vi "Begin.vi"(8 "error in":errorcluster) -> (0 "error out":errorcluster)   [LabVIEW 2018]
doc: "Called before other user functions, this VI is expected to open initial I/O refnums, load in file data, and do all program initialization. Notice that the <B>error out</B> terminal is simply used for data flow. Wiring it to other structures or subVIs ensures that this VI runs first."
uses:
  <vilib>/Rock Robotics/SystemInterfaces/DIO/FPGA_DIOPWMChannel.ctl
  <vilib>/Rock Robotics/WPI/DriverStation/WPI_DriverStationRobotMode2.ctl
  <vilib>/Rock Robotics/WPI/Joystick/WPI_JoystickDeviceEnum.ctl
  <vilib>/Rock Robotics/WPI/Solenoid/WPI_SolenoidChannel.ctl
  <vilib>/Rock Robotics/SystemInterfaces/DIO/FPGA_DIOChannel.ctl
  <vilib>/Rock Robotics/WPI/SafetyOutput/WPI_SafetyOutputConfigMenu.ctl
  Robot Global Data.vi
  <vilib>/Rock Robotics/Network Tables/NT Write String Array.vi
  <vilib>/Rock Robotics/WPI/RobotDrive/WPI_RobotDriveOpen4MotorWithTalonSRX.vi
  <vilib>/Rock Robotics/WPI/Solenoid/WPI_SolenoidOpenSingle.vi
  <vilib>/Rock Robotics/WPI/Switch/WPI_SwitchOpenLimit.vi
  <vilib>/Rock Robotics/WPI/MotorControl/WPI_MotorControlOpen TalonSRX.vi
  Global 1.vi
  <vilib>/Rock Robotics/WPI/Counter/WPI_CounterDigitalInputToDigitalSource.vi
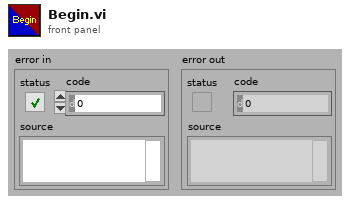
[diagram p1: front panel]
types:
  T1 = typedef "FPGA_DIOChannel.ctl" = enum8{"DIO 0", "DIO 1", "DIO 2", "DIO 3", "DIO 4", "DIO 5", "DIO 6", "DIO 7", "DIO 8", "DIO 9", "DIO MXP 0", "DIO MXP 1", "DIO MXP 2", "DIO MXP 3", "DIO MXP 4", "DIO MXP 5", "DIO MXP 6", "DIO MXP 7", "DIO MXP 8", "DIO MXP 9", "DIO MXP 10", "DIO MXP 11", "DIO MXP 12", "DIO MXP 13", "DIO MXP 14", "DIO MXP 15", "SPI Port CS1", "SPI Port CS2", "SPI Port CS3", "SPI Port MISO", "SPI Port MOSI", "Invalid"}
  T2 = typedef "WPI_SafetyOutputConfigMenu.ctl" = enum16{"Enable", "Disable"}
  T3 = typedef "FPGA_DIOPWMChannel.ctl" = enum8{"PWM 0", "PWM 1", "PWM 2", "PWM 3", "PWM 4", "PWM 5", "PWM 6", "PWM 7", "PWM 8", "PWM 9", "PWM MXP 0", "PWM MXP 1", "PWM MXP 2", "PWM MXP 3", "PWM MXP 4", "PWM MXP 5", "PWM MXP 6", "PWM MXP 7", "PWM MXP 8", "PWM MXP 9", "Invalid"}
  T4 = typedef "WPI_JoystickDeviceEnum.ctl" = enum16{"USB 0", "USB 1", "USB 2", "USB 3", "USB 4", "USB 5"}
  T5 = typedef "WPI_SolenoidChannel.ctl" = enum8{"Solenoid 0", "Solenoid 1", "Solenoid 2", "Solenoid 3", "Solenoid 4", "Solenoid 5", "Solenoid 6", "Solenoid 7", "Invalid"}
  T6 = typedef "WPI_DriverStationRobotMode2.ctl" = enum16{"Autonomous Disabled", "Autonomous Enabled", "Teleop Disabled", "Teleop Enabled", "Disconnected", "Finish", "Test Disabled", "Test Enabled", "Emergency Stopped"}
  T7 = typedef "WPI_MotorControlDeviceRef.ctl" = cluster{"DeviceStatus":errorcluster, "Type":T8, "PWM":cluster{"PWM Channel":T3, "DeadBand":T9}, "CAN":cluster{"Device Number":u8, "SetOutput VI Ref":variant, "GetOutput VI Ref":variant, "Enable VI Ref":variant, "Disable VI Ref":variant, "Data":variant}, "Invert":bool, "DIO PWM":cluster{"PWM \"Enable\" Channel":T3, "DIOChannel":T1, "PWM Rate":dbl}}
  T8 = typedef "WPI_MotorControlType.ctl" = enum16{"PWM", "CAN", "DIO PWM"}
  T9 = typedef "WPI_PWMDeadband.ctl" = cluster{"Name":string, "maxPositivePwm":i32, "minPositivePwm":i32, "centerPwm":i32, "maxNegativePwm":i32, "minNegativePwm":i32, "angularRange":u16}
  T10 = typedef "WPI_RobotDriveDevRef.ctl" = cluster{"DevStatus":errorcluster, "Motors[]":T7[], "Square Inputs":bool, "Max Output":dbl}
  T11 = typedef "WPI_JoystickDevRef.ctl" = cluster{"Device":T4}
  T12 = typedef "WPI_DigitalInputDevRef.ctl" = cluster{"DevStatus":errorcluster, "DIO Channel":T1}
  T13 = typedef "FPGA_CounterEncoderSourceConvertionLVSourceType.ctl" = cluster{"DevStatus":errorcluster, "AnalogTriggerMode?":bool, "DigitalMode":cluster{"DIO Channel":T14}, "AnalogTriggerMode":cluster{"AnalogTriggerIndex":T15, "OutputType":T16}}
  T14 = typedef "FPGA_DIODigitalSourceChannel.ctl" = enum8{"DIO 0", "DIO 1", "DIO 2", "DIO 3", "DIO 4", "DIO 5", "DIO 6", "DIO 7", "DIO 8", "DIO 9", "DIO MXP 0", "DIO MXP 1", "DIO MXP 2", "DIO MXP 3", "DIO MXP 4", "DIO MXP 5", "DIO MXP 6", "DIO MXP 7", "DIO MXP 8", "DIO MXP 9", "DIO MXP 10", "DIO MXP 11", "DIO MXP 12", "DIO MXP 13", "DIO MXP 14", "DIO MXP 15", "SPI Port CS1", "SPI Port CS2", "SPI Port CS3", "SPI Port MISO", "SPI Port MOSI", "Disabled"}
  T15 = typedef "FPGA_AnalogTriggerIndex.ctl" = enum8{"Trig 0", "Trig 1", "Trig 2", "Trig 3", "Trig 4", "Trig 5", "Trig 6", "Trig 7", "Invalid"}
  T16 = typedef "FPGA_AnalogTriggerOutType.ctl" = enum16{"InWindow", "TriggerState", "Rising", "Falling"}
  T17 = typedef "WPI_SolenoidDevRef.ctl" = cluster{"DevStatus":errorcluster, "Pneumatics Control Module":u8, "Forward Solenoid Channel":T5, "Reverse Solenoid Channel":T5}
  T18 = typedef "WPI_EncoderDevRef.ctl" = cluster{"DevStatus":errorcluster, "EncoderIndex":T19, "CounterIndex":T20, "DistancePerCount":dbl, "Decoding Type":T21}
  T19 = typedef "FPGA_EncoderIdx.ctl" = enum8{"Enc 0", "Enc 1", "Enc 2", "Enc 3", "Enc 4", "Enc 5", "Enc 6", "Enc 7", "Invalid"}
  T20 = typedef "FPGA_CounterCtrSystemIndex.ctl" = enum8{"Ctr 0", "Ctr 1", "Ctr 2", "Ctr 3", "Ctr 4", "Ctr 5", "Ctr 6", "Ctr 7", "Invalid"}
  T21 = typedef "WPI_EncoderType.ctl" = enum16{"1x", "2x", "4x"}
  T22 = typedef "WPI_SwitchDevRef.ctl" = cluster{"DevStatus":errorcluster, "DIO Channel":T1, "CntIndex":T20, "Normally Closed":bool}
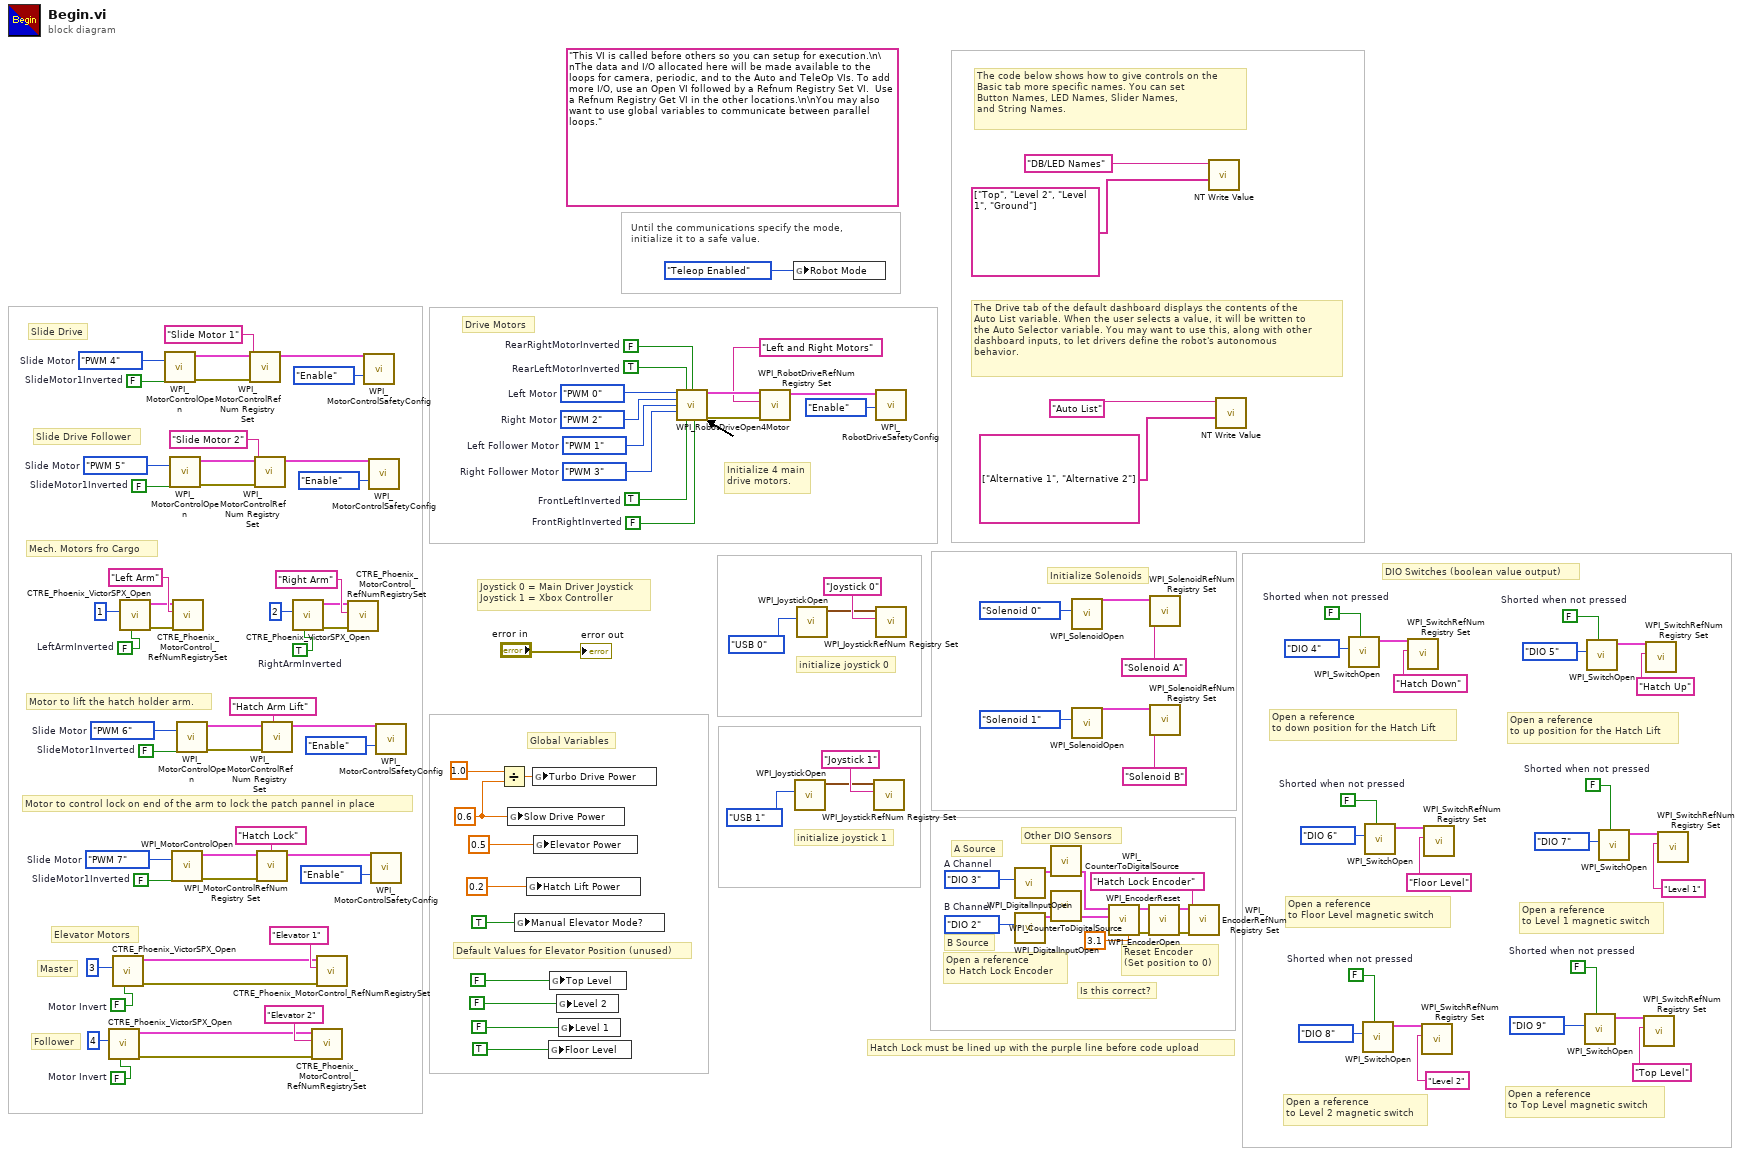
[diagram p0: block diagram]
diagram:
  w19 = FPGA_DIOChannel."DIO 2"  # B Channel
  w18 = FPGA_DIOChannel."DIO 3"  # A Channel
  w21 = FALSE  # Shorted when not pressed
  w25 = FALSE  # Shorted when not pressed
  w31 = FALSE  # SlideMotor1Inverted
  w36 = FPGA_DIOPWMChannel."PWM 7"  # Slide Motor
  w38 = FALSE  # SlideMotor1Inverted
  w43 = FPGA_DIOPWMChannel."PWM 6"  # Slide Motor
  w1 = FALSE  # Motor Invert
  w54 = FALSE  # SlideMotor1Inverted
  w60 = FPGA_DIOPWMChannel."PWM 5"  # Slide Motor
  w53 = TRUE  # RightArmInverted
  w49 = FALSE  # LeftArmInverted
  w63 = 0.6
  w44 = FALSE  # Motor Invert
  w73 = FALSE  # Shorted when not pressed
  w76 = FALSE  # SlideMotor1Inverted
  w82 = FPGA_DIOPWMChannel."PWM 4"  # Slide Motor
  w85 = FALSE  # Shorted when not pressed
  w86 = FALSE  # Shorted when not pressed
  w87 = FALSE  # Shorted when not pressed
  w104 = TRUE  # FrontLeftInverted
  w105 = FALSE  # FrontRightInverted
  w106 = FPGA_DIOPWMChannel."PWM 3"  # Right Follower Motor
  w107 = FPGA_DIOPWMChannel."PWM 1"  # Left Follower Motor
  (unwired) "This VI is called before others so you can setup for execution.\n\nThe data and I/O allocated here will be made available to the loops for camera, periodic, and to the Auto and TeleOp VIs. To add more I/O, use an Open VI followed by a Refnum Registry Set VI.  Use a Refnum Registry Get VI in the other locations.\n\nYou may also want to use global variables to communicate between parallel loops."
  w119 = FPGA_DIOPWMChannel."PWM 2"  # Right Motor
  w120 = FPGA_DIOPWMChannel."PWM 0"  # Left Motor
  w124 = TRUE  # RearLeftMotorInverted
  w125 = FALSE  # RearRightMotorInverted
  # "B Source"
  # "A Source"
  # "Hatch Lock must be lined up with the purple line before code upload"
  # "Is this correct?"
  # "Reset Encoder\n(Set position to 0)"
  # "Open a reference\nto Hatch Lock Encoder"
  # "Other DIO Sensors"
  # "DIO Switches (boolean value output)"
  # "Open a reference\nto up position for the Hatch Lift"
  # "Open a reference\nto down position for the Hatch Lift"
  # "Default Values for Elevator Position (unused)"
  # "Elevator Motors"
  # "Motor to control lock on end of the arm to lock the patch pannel in place"
  # "Motor to lift the hatch holder arm."
  # "Global Variables"
  # "Follower"
  # "Master"
  # "Slide Drive Follower"
  # "Slide Drive"
  # "Open a reference\nto Top Level magnetic switch"
  # "Drive Motors"
  # "Mech. Motors fro Cargo"
  # "Open a reference\nto Level 2 magnetic switch"
  # "Open a reference\nto Level 1 magnetic switch"
  # "Open a reference\nto Floor Level magnetic switch"
  # "Initialize Solenoids"
  # "Initialize 4 main\ndrive motors."
  # "Joystick 0 = Main Driver Joystick\nJoystick 1 = Xbox Controller"
  # "initialize joystick 1"
  # "The Drive tab of the default dashboard displays the contents of the\nAuto List variable. When the user selects a value, it will be written to\nthe Auto Selector variable. You may want to use this, along with other\ndashboard inputs, to let drivers define the robot's autonomous\nbehavior."
  # "The code below shows how to give controls on the\nBasic tab more specific names. You can set\nButton Names, LED Names, Slider Names,\nand String Names."
  # "initialize joystick 0"
  # "Until the communications specify the mode,\ninitialize it to a safe value."
  n1 = call <vilib>:"CTRE_Phoenix_VictorSPX_Open.vi"("Invert"=w1, "Device Number"=u8 4) -> ("error out"=w4:errorcluster, "CAN Talon SRX Ref"=w3:T7)  [unwired: 8 in]
  n2 = call <vilib>:"CTRE_Phoenix_VictorSPX_Open.vi"("Invert"=w44, "Device Number"=u8 3) -> ("error out"=w5:errorcluster, "CAN Talon SRX Ref"=w6:T7)  [unwired: 8 in]
  n3 = call <vilib>:"CTRE_Phoenix_VictorSPX_Open.vi"("Invert"=w49, "Device Number"=u8 1) -> ("error out"=w46:errorcluster, "CAN Talon SRX Ref"=w47:T7)  [unwired: 8 in]
  n4 = call-poly <vilib>:"WPI_MotorControlOpen.vi"("Invert"=w76, "PWM Channel"=w82) -> ("error out"=w80:errorcluster, "MotorControlDeviceRef"=w81:T7)  [unwired: 8 in]
  n5 = call-poly <vilib>:"WPI_MotorControlOpen.vi"("Invert"=w54, "PWM Channel"=w60) -> ("error out"=w58:errorcluster, "MotorControlDeviceRef"=w59:T7)  [unwired: 8 in]
  n6 = call-poly <vilib>:"WPI_MotorControlOpen.vi"("Invert"=w31, "PWM Channel"=w36) -> ("error out"=w34:errorcluster, "MotorControlDeviceRef"=w35:T7)  [unwired: 8 in]
  n7 = call <vilib>:"CTRE_Phoenix_MotorControl_RefNumRegistrySet.vi"("error in (no error)"=w46, "refnum name"="Left Arm", "PhoenixMotorControlDevRef"=w47) -> ()  [unwired: 7 in, 2 out]
  n8 = call-poly <vilib>:"WPI_MotorControlOpen.vi"("Invert"=w38, "PWM Channel"=w43) -> ("error out"=w41:errorcluster, "MotorControlDeviceRef"=w42:T7)  [unwired: 8 in]
  n9 = call <vilib>:"WPI_MotorControlRefNum Registry Set.vi"("error in (no error)"=w80, "refnum name"="Slide Motor 1", "MotorControlDevRef"=w81) -> ("MotorControlDevRef"=w78:T7)  [unwired: 7 in, 1 out]
  n10 = call <vilib>:"WPI_MotorControlRefNum Registry Set.vi"("error in (no error)"=w58, "refnum name"="Slide Motor 2", "MotorControlDevRef"=w59) -> ("MotorControlDevRef"=w56:T7)  [unwired: 7 in, 1 out]
  n11 = call <vilib>:"WPI_MotorControlRefNum Registry Set.vi"("error in (no error)"=w34, "refnum name"="Hatch Lock", "MotorControlDevRef"=w35) -> ("MotorControlDevRef"=w33:T7)  [unwired: 7 in, 1 out]
  n12 = call <vilib>:"WPI_MotorControlRefNum Registry Set.vi"("error in (no error)"=w41, "refnum name"="Hatch Arm Lift", "MotorControlDevRef"=w42) -> ("MotorControlDevRef"=w40:T7)  [unwired: 7 in, 1 out]
  n13 = call <vilib>:"CTRE_Phoenix_VictorSPX_Open.vi"("Invert"=w53, "Device Number"=u8 2) -> ("error out"=w50:errorcluster, "CAN Talon SRX Ref"=w51:T7)  [unwired: 8 in]
  n14 = call <vilib>:"CTRE_Phoenix_MotorControl_RefNumRegistrySet.vi"("error in (no error)"=w4, "refnum name"="Elevator 2", "PhoenixMotorControlDevRef"=w3) -> ()  [unwired: 7 in, 2 out]
  n15 = call <vilib>:"CTRE_Phoenix_MotorControl_RefNumRegistrySet.vi"("error in (no error)"=w5, "refnum name"="Elevator 1", "PhoenixMotorControlDevRef"=w6) -> ()  [unwired: 7 in, 2 out]
  n16 = call <vilib>:"CTRE_Phoenix_MotorControl_RefNumRegistrySet.vi"("error in (no error)"=w50, "refnum name"="Right Arm", "PhoenixMotorControlDevRef"=w51) -> ()  [unwired: 7 in, 2 out]
  n17 = call <vilib>:"WPI_MotorControlSafetyConfig.vi"("mode"=WPI_SafetyOutputConfigMenu."Enable", "MotorControlDevRef"=w78) -> ()  [unwired: 8 in, 2 out]
  n18 = call <vilib>:"WPI_MotorControlSafetyConfig.vi"("mode"=WPI_SafetyOutputConfigMenu."Enable", "MotorControlDevRef"=w56) -> ()  [unwired: 8 in, 2 out]
  n19 = call <vilib>:"WPI_MotorControlSafetyConfig.vi"("mode"=WPI_SafetyOutputConfigMenu."Enable", "MotorControlDevRef"=w33) -> ()  [unwired: 8 in, 2 out]
  n20 = call <vilib>:"WPI_MotorControlSafetyConfig.vi"("mode"=WPI_SafetyOutputConfigMenu."Enable", "MotorControlDevRef"=w40) -> ()  [unwired: 8 in, 2 out]
  n21 = Divide(x=1.0, y=w63) -> (x/y=w69:dbl)
  n22 = global write "Global 1.vi" "Slow Drive Power"(w63) -> ()
  n23 = global write "Global 1.vi" "Manual Elevator Mode?"(TRUE) -> ()
  n24 = global write "Global 1.vi" "Hatch Lift Power"(0.2) -> ()
  n25 = global write "Global 1.vi" "Turbo Drive Power"(w69) -> ()
  n26 = global write "Global 1.vi" "Elevator Power"(0.5) -> ()
  n27 = global write "Global 1.vi" "Floor Level"(TRUE) -> ()
  n28 = global write "Global 1.vi" "Top Level"(FALSE) -> ()
  n29 = global write "Global 1.vi" "Level 2"(FALSE) -> ()
  n30 = global write "Global 1.vi" "Level 1"(FALSE) -> ()
  n31 = call-poly <vilib>:"WPI_RobotDriveOpen4Motor.vi"("Rear Left Motor"=w120, "Rear Left Motor Inverted"=w124, "Rear Right Motor Inverted"=w125, "Rear Right Motor"=w119, "Front Left Motor"=w107, "Front Right Motor"=w106, "Front Left Motor Inverted"=w104, "Front Right Motor Inverted"=w105) -> ("RobotDriveDevRef"=w123:T10, "error out"=w121:errorcluster)  [unwired: 6 in]
  n32 = call <vilib>:"WPI_RobotDriveRefNum Registry Set.vi"("error in (no error)"=w121, "refnum name"="Left and Right Motors", "RobotDriveDevRef"=w123) -> ("RobotDriveDevRef"=w118:T10)  [unwired: 1 in, 7 out]
  n33 = global write "Robot Global Data.vi" "Robot Mode"(WPI_DriverStationRobotMode2."Teleop Enabled" ("Robot Mode")) -> ()
  n34 = call <vilib>:"WPI_JoystickOpen.vi"("JoystickDevice"=WPI_JoystickDeviceEnum."USB 1") -> ("JoystickDevRef"=w96:T11)  [unwired: 10 in]
  n35 = call <vilib>:"WPI_JoystickOpen.vi"("JoystickDevice"=WPI_JoystickDeviceEnum."USB 0") -> ("JoystickDevRef"=w114:T11)  [unwired: 10 in]
  n36 = call <vilib>:"WPI_JoystickRefNum Registry Set.vi"("refnum name"="Joystick 1", "JoystickDevRef"=w96) -> ()  [unwired: 8 in, 2 out]
  n37 = call <vilib>:"WPI_RobotDriveSafetyConfig.vi"("mode"=WPI_SafetyOutputConfigMenu."Enable", "RobotDriveDevRef"=w118) -> ()  [unwired: 8 in, 2 out]
  n38 = call <vilib>:"WPI_JoystickRefNum Registry Set.vi"("refnum name"="Joystick 0", "JoystickDevRef"=w114) -> ()  [unwired: 8 in, 2 out]
  n39 = call <vilib>:"WPI_DigitalInputOpen.vi"("DIO Channel"=w18) -> ("DigitalInputDevRef"=w15:T12)  [unwired: 1 in, 9 out]
  n40 = call <vilib>:"WPI_DigitalInputOpen.vi"("DIO Channel"=w19) -> ("DigitalInputDevRef"=w16:T12)  [unwired: 1 in, 9 out]
  n41 = call-poly <vilib>:"WPI_CounterToDigitalSource.vi"("DigitalInputDevRef"=w15) -> ("Digital Source"=w14:T13)  [unwired: 6 out]
  n42 = call-poly <vilib>:"WPI_CounterToDigitalSource.vi"("DigitalInputDevRef"=w16) -> ("Digital Source"=w17:T13)  [unwired: 6 out]
  n43 = call-poly <vilib>:"WPI_SolenoidOpen.vi"("Solenoid Channel"=WPI_SolenoidChannel."Solenoid 0") -> ("SolenoidDevRef"=w102:T17)  [unwired: 9 in, 1 out]
  n44 = call-poly <vilib>:"WPI_SolenoidOpen.vi"("Solenoid Channel"=WPI_SolenoidChannel."Solenoid 1") -> ("SolenoidDevRef"=w99:T17)  [unwired: 9 in, 1 out]
  n45 = call <vilib>:"WPI_EncoderOpen.vi"("DistancePerCount"=3.1, "BSource"=w17, "ASource"=w14) -> ("error out"=w11:errorcluster, "EncoderDevRef"=w10:T18)  [unwired: 5 in, 2 out]
  n46 = call <vilib>:"WPI_EncoderReset.vi"("error in (no error)"=w11, "EncoderDevRef"=w10) -> ("error out"=w8:errorcluster, "EncoderDevRef"=w9:T18)  [unwired: 8 in]
  n47 = call <vilib>:"WPI_SolenoidRefNum Registry Set.vi"("refnum name"="Solenoid A", "SolenoidDevRef"=w102) -> ()  [unwired: 8 in, 2 out]
  n48 = call <vilib>:"WPI_SolenoidRefNum Registry Set.vi"("refnum name"="Solenoid B", "SolenoidDevRef"=w99) -> ()  [unwired: 8 in, 2 out]
  n49 = call <vilib>:"WPI_EncoderRefNum Registry Set.vi"("error in (no error)"=w8, "refnum name"="Hatch Lock Encoder", "EncoderDevRef"=w9) -> ()  [unwired: 7 in, 2 out]
  n50 = call-poly <vilib>:"NT Write Value.vi"("String Array"=string[] ["Top", "Level 2", "Level 1", "Ground"], "Name"="DB/LED Names") -> ()  [unwired: 9 in, 1 out]
  n51 = call-poly <vilib>:"NT Write Value.vi"("String Array"=string[] ["Alternative 1", "Alternative 2"], "Name"="Auto List") -> ()  [unwired: 9 in, 1 out]
  n52 = call-poly <vilib>:"WPI_SwitchOpen.vi"("Normally Closed"=w25, "DIO Channel"=FPGA_DIOChannel."DIO 4") -> ("SwitchDevRef"=w28:T22)  [unwired: 8 in, 1 out]
  n53 = call-poly <vilib>:"WPI_SwitchOpen.vi"("Normally Closed"=w85, "DIO Channel"=FPGA_DIOChannel."DIO 8") -> ("SwitchDevRef"=w90:T22)  [unwired: 8 in, 1 out]
  n54 = call-poly <vilib>:"WPI_SwitchOpen.vi"("Normally Closed"=w87, "DIO Channel"=FPGA_DIOChannel."DIO 6") -> ("SwitchDevRef"=w94:T22)  [unwired: 8 in, 1 out]
  n55 = call <vilib>:"WPI_SwitchRefNum Registry Set.vi"("refnum name"="Hatch Down", "SwitchDevRef"=w28) -> ()  [unwired: 8 in, 2 out]
  n56 = call <vilib>:"WPI_SwitchRefNum Registry Set.vi"("refnum name"="Level 2", "SwitchDevRef"=w90) -> ()  [unwired: 8 in, 2 out]
  n57 = call <vilib>:"WPI_SwitchRefNum Registry Set.vi"("refnum name"="Floor Level", "SwitchDevRef"=w94) -> ()  [unwired: 8 in, 2 out]
  n58 = call-poly <vilib>:"WPI_SwitchOpen.vi"("Normally Closed"=w73, "DIO Channel"=FPGA_DIOChannel."DIO 9") -> ("SwitchDevRef"=w75:T22)  [unwired: 8 in, 1 out]
  n59 = call-poly <vilib>:"WPI_SwitchOpen.vi"("Normally Closed"=w21, "DIO Channel"=FPGA_DIOChannel."DIO 5") -> ("SwitchDevRef"=w24:T22)  [unwired: 8 in, 1 out]
  n60 = call-poly <vilib>:"WPI_SwitchOpen.vi"("Normally Closed"=w86, "DIO Channel"=FPGA_DIOChannel."DIO 7") -> ("SwitchDevRef"=w92:T22)  [unwired: 8 in, 1 out]
  n61 = call <vilib>:"WPI_SwitchRefNum Registry Set.vi"("refnum name"="Top Level", "SwitchDevRef"=w75) -> ()  [unwired: 8 in, 2 out]
  n62 = call <vilib>:"WPI_SwitchRefNum Registry Set.vi"("refnum name"="Hatch Up", "SwitchDevRef"=w24) -> ()  [unwired: 8 in, 2 out]
  n63 = call <vilib>:"WPI_SwitchRefNum Registry Set.vi"("refnum name"="Level 1", "SwitchDevRef"=w92) -> ()  [unwired: 8 in, 2 out]
  "error out" <- "error in"
